vi "Initialize.vi"(8 "error in":errorcluster, 11 "Plugin in":refnum<class "Dynamic Channel.lvclass">) -> (0 "error out":errorcluster, 3 "Plugin out":refnum<class "Dynamic Channel.lvclass">)   [LabVIEW 2020, in "Dynamic Channel.lvlib" / "Dynamic Channel.lvclass"]
uses:
  Dynamic Channel.lvclass
  <vilib>/FlexLogger/SDK/PluginSDK.lvlibp/PEFClasses/SDK/Plugin/Plugin.lvclass
  <vilib>/FlexLogger/SDK/PluginSDK.lvlibp/PEFClasses/SDK/Plugin/ParameterAccess/Write I32.vi
  Dynamic Channel Global.vi
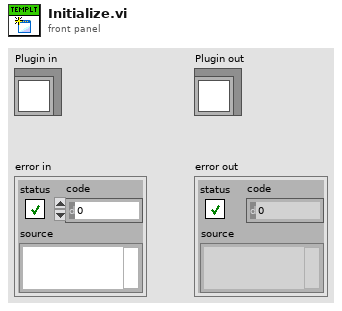
[diagram p1: front panel]
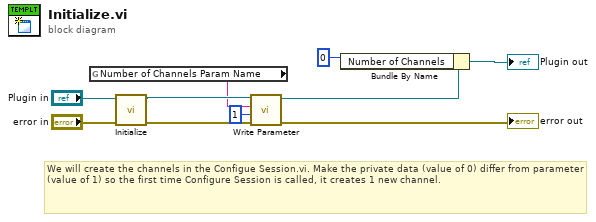
[diagram p0: block diagram]
diagram:
  # "We will create the channels in the Configue Session.vi. Make the private data (value of 0) differ from parameter (value of 1) so the first time Configure Session is called, it creates 1 new channel."
  n1 = global read "Dynamic Channel Global.vi" "Number of Channels Param Name"() -> (w1:string)
  n2 = call-parent "Initialize.vi"("error in (no error)"="error in", "Plugin in"="Plugin in") -> ("error out"=w7:errorcluster, "Plugin out"=w8:refnum<class "Dynamic Channel.lvclass">)  [unwired: 8 in]
  n3 = call-poly <vilib>:"Write Parameter.vi"("error in (no error)"=w7, "Value"=1, "Name"=w1, "Plugin in"=w8) -> ("error out"=→"error out":errorcluster, "Plugin out"=w6:refnum<class "Dynamic Channel.lvclass">)  [unwired: 6 in]
  n4 = Bundle By Name(cluster=w6, "Number of Channels"=u32 0) -> (→"Plugin out":refnum<class "Dynamic Channel.lvclass">)
